vi "NAND.vi"() -> ()   [LabVIEW 2013]
panel:
  out "Boolean 4":bool
  in  "Boolean 3":bool
  in  "Boolean 2":bool
  in  "Boolean":bool
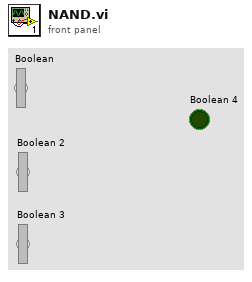
[diagram p1: front panel]
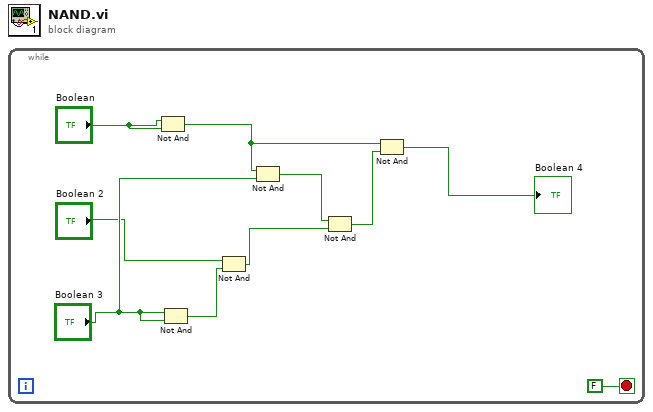
[diagram p0: block diagram]
diagram:
  n1 = while {
    stop <- FALSE stop-if-true
    n2 = Not And(1:"Boolean", 2:"Boolean") -> (0:w1:bool)
    n3 = Not And(1:"Boolean 3", 2:"Boolean 3") -> (0:w3:bool)
    n4 = Not And(1:w3, 2:"Boolean 2") -> (0:w8:bool)
    n5 = Not And(1:"Boolean 3", 2:w1) -> (0:w9:bool)
    n6 = Not And(1:w8, 2:w9) -> (0:w6:bool)
    n7 = Not And(1:w6, 2:w1) -> (0:→"Boolean 4":bool)
  }
